vi "Write value range.vi"(8 "error in (no error)":errorcluster, 10 "value range":string(combo)="Omit", 11 "DAQNavi_AO in":refnum<class "DAQNavi_AO.lvclass">) -> (0 "error out":errorcluster, 3 "DAQNavi_AO out":refnum<class "DAQNavi_AO.lvclass">)   [LabVIEW 2021, in "DAQNavi_AO.lvclass"]
uses:
  DAQNavi_AO.lvclass
  DAQNavi_AO.lvclass/DAQNavi_AO.ctl
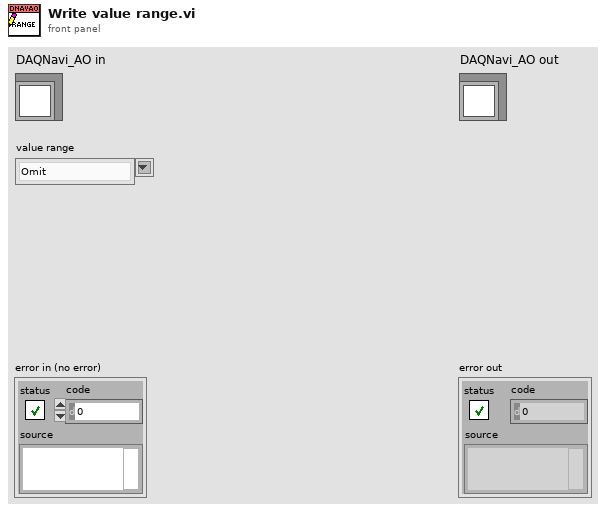
[diagram p1: front panel]
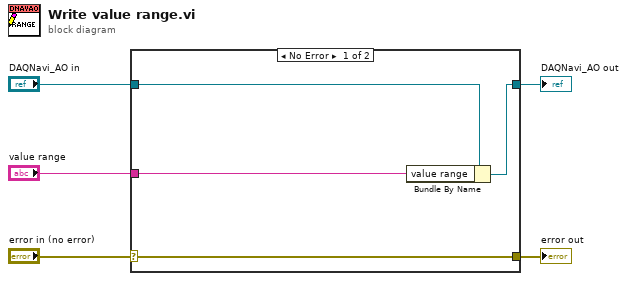
[diagram p0: block diagram]
diagram:
  n1 = case shown="No Error" "error in (no error)" {
    selector: "error in (no error)" -> [w9 w10]
    tunnel: [w9 w10] -> w4
    tunnel: [w7 w11] -> w2
    tunnel: "DAQNavi_AO in" -> [w8 w11]
    tunnel: "value range" -> [w6 _]
    frame No Error {
      n2 = Bundle By Name(cluster=w8, "value range"=w6) -> (w7:refnum<class "DAQNavi_AO.lvclass">)
    }
    frame Error {
    }
  }
  "error out" <- w4
  "DAQNavi_AO out" <- w2
